vi "set Start and Stop Frequency.vi"(8 "error in (no error)":errorcluster, 10 "Start/Stop Frequency(Hz)":T1 {"Stop" format="%#_6p"; "Start" format="%#_6p"}, 11 "FSV-40N in":refnum<class "FSV-40N.lvclass">) -> (0 "error out":errorcluster, 3 "FSV-40N out":refnum<class "FSV-40N.lvclass">)   [LabVIEW 2023, in "Spectrum Analyzer.lvlib" / "FSV-40N.lvclass"]
uses:
  FSV-40N.lvclass
  TYPE DEFINITION/TYPE Start and Stop Frequency.ctl
  FSV-40N.lvclass/FSV-40N.ctl
  Spectrum Analyzer.lvlib
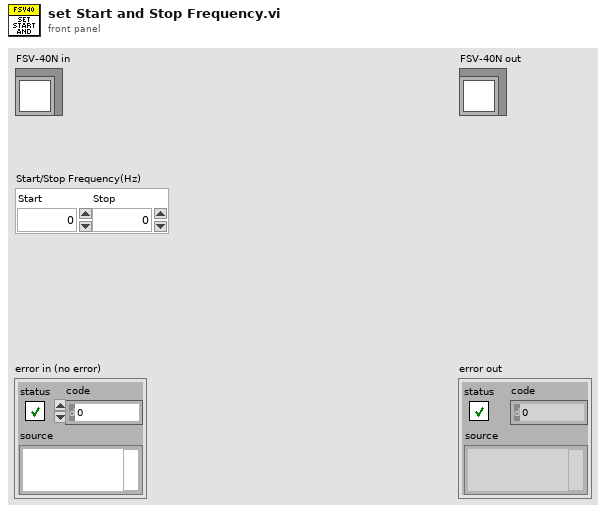
[diagram p1: front panel]
types:
  T1 = typedef "Spectrum Analyzer.lvlib/TYPE Start and Stop Frequency.ctl" = cluster{"Start":dbl, "Stop":dbl}
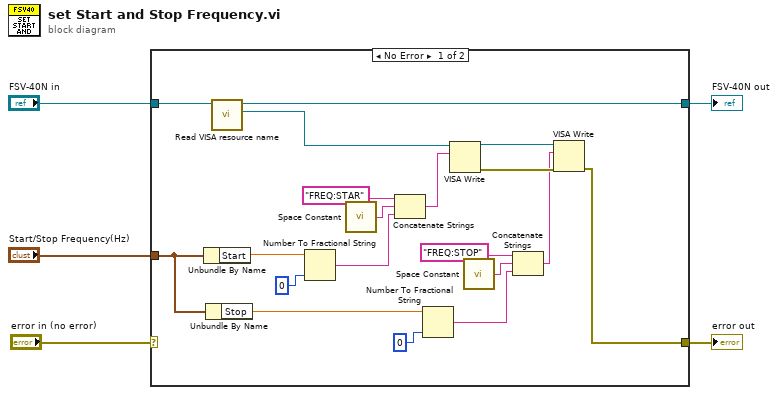
[diagram p0: block diagram]
diagram:
  n1 = case shown="No Error" "error in (no error)" {
    selector: "error in (no error)" -> [_ w26]
    tunnel: "FSV-40N in" -> [w24 w25]
    tunnel: [w6 w26] -> w3
    tunnel: [w7 w25] -> w2
    tunnel: "Start/Stop Frequency(Hz)" -> [w14 _]
    frame No Error {
      n2 = Unbundle By Name(w14) -> ("Start"=w20:dbl)
      n3 = Unbundle By Name(w14) -> ("Stop"=w9:dbl)
      n4 = call "Read VISA resource name.vi"("FSV-40N in"=w24) -> ("VISA resource name"=w23:refnum<visa-resource-name>, "FSV-40N out"=w7:refnum<class "FSV-40N.lvclass">)  [unwired: 8 in, 1 out]
      n5 = Number To Fractional String(number=w20, precision (6)=i16 0) -> (F-format string=w18:string)  [unwired: 2 in]
      n6 = call <vilib>:"Space Constant.vi"() -> ("String"=w21:string)
      n7 = Concatenate Strings("FREQ:STAR", w21, w18) -> (w17:string)
      n8 = Number To Fractional String(number=w9, precision (6)=i16 0) -> (F-format string=w13:string)  [unwired: 2 in]
      n9 = VISA Write(VISA resource name=w23, write buffer=w17) -> (VISA resource name out=w16:refnum<visa-resource-name>, error out=w15:errorcluster)  [unwired: 1 in, 1 out]
      n10 = call <vilib>:"Space Constant.vi"() -> ("String"=w11:string)
      n11 = Concatenate Strings("FREQ:STOP", w11, w13) -> (w8:string)
      n12 = VISA Write(VISA resource name=w16, write buffer=w8, error in (no error)=w15) -> (error out=w6:errorcluster)  [unwired: 2 out]
    }
    frame Error {
    }
  }
  "error out" <- w3
  "FSV-40N out" <- w2
